vi "Test Helper Loop.vi"(8 "error in (no error)":errorcluster, 11 "Helper Loop Test In":refnum<class "Helper Loop Test.lvclass">) -> (0 "error out":errorcluster, 3 "Helper Loop Test Out":refnum<class "Helper Loop Test.lvclass">)   [LabVIEW 2020, in "Helper Loop Test.lvclass"]
uses:
  Helper Loop Test.lvclass
  C:/Program Files (x86)/National Instruments/LabVIEW 2020/vi.lib/Astemes/LUnit/Test Case.lvclass
  source/Framework Test Suite/Mock Process/Mock Process.lvclass
  C:/git/astemes-triarc-framework/source/Framework/Process/Process.lvclass
  <vilib>/Astemes/LUnit/Test Case.lvclass/Test Case.ctl
  source/Framework/Process/Process.lvclass/Process.ctl
  940a0d52-585f-4e02-8690-06099146145a.vi
  source/Framework/Broadcast Event Dequeuers/Execution timer.vi
  <vilib>/Astemes/LUnit/Append Pass Result.vi
  <vilib>/Astemes/LUnit/Append Fail Result.vi
  940a0d52-585f-4e02-8690-06099146145a.vi/9c5d11cd-9439-4240-a1ee-d9baace9c924.vi
  source/Framework/Process/Private/SubVIs/Wait for finish.vi
  source/Framework/Process/Private/SubVIs/Set Lifecycle State.vi
  source/Framework/Process/Protected/Messaging/Send Message.vi
  <vilib>/Astemes/LUnit/Run In UI.vi
  source/Framework/Process/Private/SubVIs/Handle Debug Data.vi
  <vilib>/Utility/error.llb/Clear Errors.vi
  source/Framework/Logging/Log Debug.vi
  <vilib>/AdvancedString/1D String Array to Delimited String.vi
  <vilib>/Utility/High Resolution Relative Seconds.vi
  source/Framework/Broadcast Event Dequeuers/Dequeue Broadcast Message.vi
  source/Framework/Process/Public/Lifecycle/Get Lifecycle State.vi
  <vilib>/Utility/error.llb/Error Cluster From Error Code.vi
  source/Framework/Process/Public/Read Name.vi
  source/Framework/Callback/Callback.lvclass
  source/Framework/Process/Process.lvclass
  Helper Loop Test.lvclass/Helper Loop Test.ctl
  <vilib>/Astemes/LUnit/Test Case.lvclass
  source/Framework/Broadcast Event Dequeuers/Broadcast Event Dequeuers.lvlib
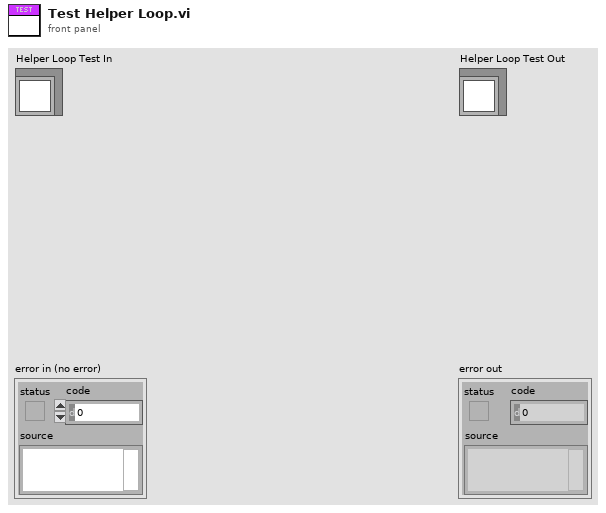
[diagram p1: front panel]
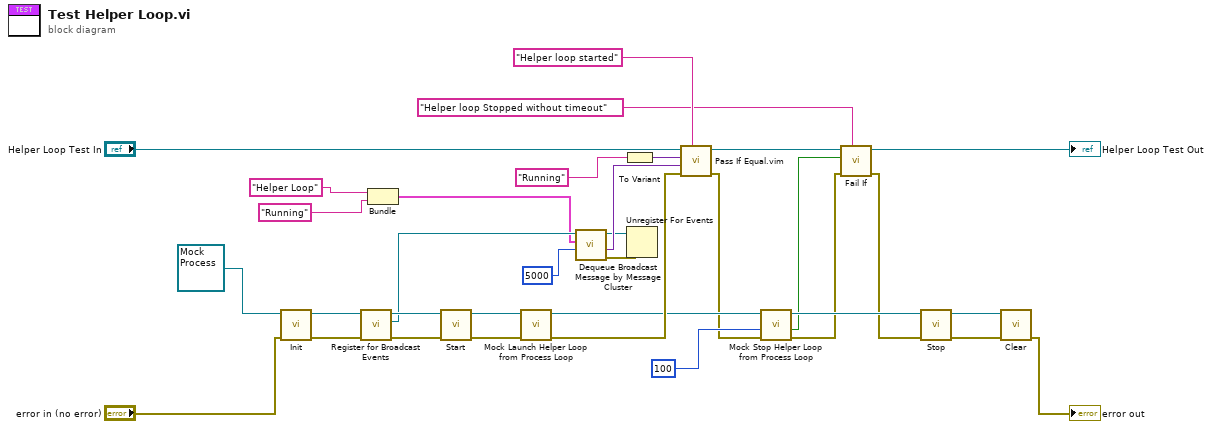
[diagram p0: block diagram]
diagram:
  n1 = call-dynamic "Init.vi"("error in (no error)"="error in (no error)", "Mock Process In"=refnum<class "Mock Process.lvclass"> refnum) -> ("error out"=w32:errorcluster, "Mock Process Out"=w33:refnum<class "Mock Process.lvclass">)  [unwired: 8 in]
  n2 = call "Register for Broadcast Events.vi"("error in (no error)"=w32, "Process In"=w33) -> ("error out"=w30:errorcluster, "Event Registration Refnum Out"=w7:refnum<event-registration>, "Process Out"=w31:refnum<class "Mock Process.lvclass">)  [unwired: 7 in]
  n3 = Bundle("y"="Helper Loop", "Description"="Running") -> (w2:cluster{"y":string, "Description":string})  [unwired: 1 in]
  n4 = call "Start.vi"("error in (no error)"=w30, "Process In"=w31) -> ("error out"=w28:errorcluster, "Process Out"=w29:refnum<class "Mock Process.lvclass">)  [unwired: 7 in, 1 out]
  n5 = call "Mock Launch Helper Loop from Process Loop.vi"("error in (no error)"=w28, "Mock Process in"=w29) -> ("error out"=w19:errorcluster, "Mock Process out"=w18:refnum<class "Mock Process.lvclass">)  [unwired: 8 in]
  n6 = call "Dequeue Broadcast Message by Message Cluster.vi"("Timeout (-1)"=5000, "Message"=w2, "Event Registration Refnum"=w7) -> ("error out"=w6:errorcluster, "Message Data"=w8:variant, "Event Registration Refnum Out"=w5:refnum<event-registration>)  [unwired: 4 in, 2 out]
  n7 = To Variant(anything="Running") -> (Variant=w1:variant)
  n8 = Unregister For Events(event registration refnum=w5, error in=w6) -> ()  [unwired: 1 out]
  n9 = call "Pass If Equal.vim"("Description"="Helper loop started", "error in (no error)"=w19, "Actual"=w8, "Expected"=w1, "LUnit Test Case In"="Helper Loop Test In") -> ("error out"=w16:errorcluster, "LUnit Test Case Out"=w24:refnum<class "Helper Loop Test.lvclass">)  [unwired: 5 in]
  n10 = call "Mock Stop Helper Loop from Process Loop.vi"("error in (no error)"=w16, "timeout in ms (-1)"=100, "Mock Process in"=w18) -> ("error out"=w13:errorcluster, "timed out?"=w15:bool, "Mock Process out"=w27:refnum<class "Mock Process.lvclass">)  [unwired: 6 in]
  n11 = call <vilib>:"Fail If.vi"("Description"="Helper loop Stopped without timeout", "error in (no error)"=w13, "Fail?"=w15, "LUnit Test Case In"=w24) -> ("error out"=w12:errorcluster, "LUnit Test Case Out"=→"Helper Loop Test Out":refnum<class "Helper Loop Test.lvclass">)  [unwired: 6 in]
  n12 = call "Stop.vi"("error in (no error)"=w12, "Process In"=w27) -> ("error out"=w26:errorcluster, "Process Out"=w11:refnum<class "Mock Process.lvclass">)  [unwired: 7 in, 1 out]
  n13 = call-dynamic "Clear.vi"("error in (no error)"=w26, "Mock Process In"=w11) -> ("error out"=→"error out":errorcluster)  [unwired: 9 in]
